vi "PPL_TRAJECTORY_EXECUTE_REL.vi"(8 "Init":bool, 9 "Max Wheel Speed M/S":dbl=2.5, 11 "Gyro Heading\nRAD":dbl) -> (0 "AtReference":bool, 1 "Position Error Ft":dbl, 2 "Right Speed Dmd M/S":dbl, 3 "Left Speed Dmd M/S":dbl)   [LabVIEW 2019]
uses:
  <vilib>/Rock Robotics/WPI/ThirdParty/MJansen/PathPlanner/TypeDef/PathPlannerTrajectory.ctl
  <vilib>/Rock Robotics/WPI/ThirdParty/MJansen/PathPlanner/TypeDef/PathPlannerTrajectoryState.ctl
  <vilib>/Rock Robotics/WPI/ThirdParty/JAS_Junk/TrajLib/TypeDef/TRANSLATION2D.ctl
  <vilib>/Rock Robotics/WPI/ThirdParty/JAS_Junk/TrajLib/TypeDef/ROTATION2D.ctl
  <vilib>/Rock Robotics/WPI/ThirdParty/MJansen/PathPlanner/TypeDef/PathPlannerPathConstraints.ctl
  <vilib>/Rock Robotics/WPI/ThirdParty/JAS_Junk/TrajLib/VI/Util_GetTime_U32.vi
  <vilib>/Rock Robotics/WPI/ThirdParty/JAS_Junk/TrajLib/Conv_Deg_Radians.vi
  <vilib>/Rock Robotics/WPI/ThirdParty/JAS_Junk/TrajLib/VI/DiffDrvOdom2_New.vi
  <vilib>/Rock Robotics/WPI/ThirdParty/JAS_Junk/TrajLib/VI/DiffDrvOdom2_Reset.vi
  <vilib>/Rock Robotics/WPI/ThirdParty/JAS_Junk/TrajLib/VI/DiffDrvOdom2_Update.vi
  <vilib>/Rock Robotics/WPI/ThirdParty/JAS_Junk/TrajLib/Rotation2d_GetRadians.vi
  <vilib>/Rock Robotics/SystemInterfaces/NetworkCommunication/NetComm_UsageReport_report.vi
  <vilib>/Rock Robotics/WPI/ThirdParty/JAS_Junk/TrajLib/Pose2d_getRotation.vi
  <vilib>/Rock Robotics/WPI/ThirdParty/JAS_Junk/TrajLib/Rotation2d_Minus.vi
  <vilib>/Rock Robotics/WPI/ThirdParty/JAS_Junk/TrajLib/Rotation2d_Plus.vi
  <vilib>/Rock Robotics/WPI/ThirdParty/JAS_Junk/TrajLib/Twist2d_Create.vi
  <vilib>/Rock Robotics/WPI/ThirdParty/JAS_Junk/TrajLib/Rotation2d_UnaryMinus.vi
  <vilib>/Rock Robotics/WPI/ThirdParty/JAS_Junk/TrajLib/Rotation2d_RotateBy.vi
  <vilib>/Rock Robotics/WPI/ThirdParty/JAS_Junk/TrajLib/Rotation2d_CreateXY.vi
  <vilib>/Rock Robotics/WPI/ThirdParty/JAS_Junk/TrajLib/Util_CalcDist.vi
  <vilib>/Rock Robotics/WPI/ThirdParty/JAS_Junk/TrajLib/VI/Util_GetTime_U64.vi
  PPL_TRAJECTORY_GLOBALS.vi
  Diff_Drive_System/PPL_DRIVE_GLOBALS.vi
  <vilib>/Rock Robotics/WPI/ThirdParty/JAS_Junk/TrajLib/Globals/Util_LibraryGlobals.vi
  <vilib>/Rock Robotics/WPI/ThirdParty/JAS_Junk/TrajLib/Pose2d_Exp.vi
  <vilib>/Rock Robotics/WPI/ThirdParty/JAS_Junk/TrajLib/Trajectory_Library.lvlib
  <vilib>/Rock Robotics/WPI/ThirdParty/MJansen/PathPlanner/PathPlanner24.lvlib
panel:
  out "PathPlannerTrajectory":T1 {"States"."TargetHolonomicRotation"."SIN" format="%13.4f"; "States"."TargetHolonomicRotation"."COS" format="%13.4f"; "States"."TargetHolonomicRotation"."VALUE" format="%13.4f"; "States"."Heading"."SIN" format="%13.4f"; "States"."Heading"."COS" format="%13.4f"; "States"."Heading"."VALUE" format="%13.4f"; "States"."PositionMeters"."Y" format="%14.3f"; "States"."PositionMeters"."X" format="%14.3f"}
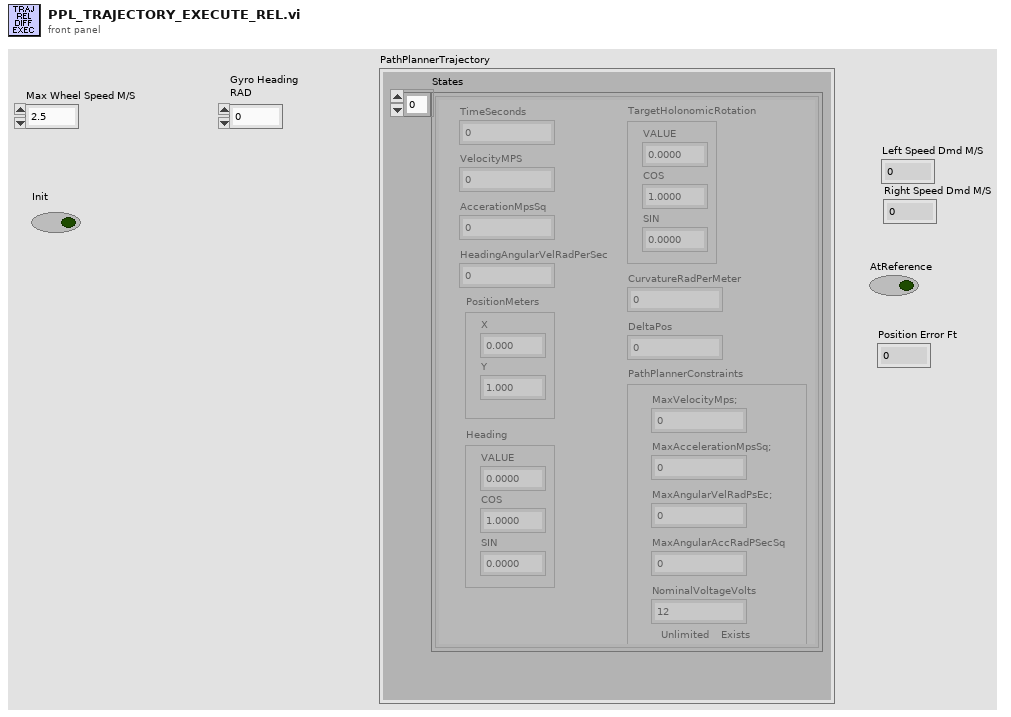
[diagram p1: front panel]
types:
  T1 = typedef "PathPlanner24.lvlib/PathPlannerTrajectory.ctl" = cluster{"States":T2[]}
  T2 = typedef "PathPlanner24.lvlib/PathPlannerTrajectoryState.ctl" = cluster{"TimeSeconds":dbl, "VelocityMPS":dbl, "AccerationMpsSq":dbl, "HeadingAngularVelRadPerSec":dbl, "PositionMeters":T3, "Heading":T4, "TargetHolonomicRotation":T4, "CurvatureRadPerMeter":dbl, "PathPlannerConstraints":T5, "DeltaPos":dbl}
  T3 = typedef "Trajectory_Library.lvlib/TRANSLATION2D.ctl" = cluster{"X":dbl, "Y":dbl}
  T4 = typedef "Trajectory_Library.lvlib/ROTATION2D.ctl" = cluster{"VALUE":dbl, "COS":dbl, "SIN":dbl}
  T5 = typedef "PathPlanner24.lvlib/PathPlannerPathConstraints.ctl" = cluster{"MaxVelocityMps;":dbl, "MaxAccelerationMpsSq;":dbl, "MaxAngularVelRadPsEc;":dbl, "MaxAngularAccRadPSecSq":dbl, "Exists":bool, "Unlimited":bool, "NominalVoltageVolts":dbl}
  T6 = typedef "Trajectory_Library.lvlib/POSE2D.ctl" = cluster{"TRANSLATION":T3, "ROTATION":T4}
  T7 = typedef "Trajectory_Library.lvlib/DIFF_DRIVE_KINEMATICS.ctl" = cluster{"TrackWidth_Meters":dbl}
  T8 = typedef "Trajectory_Library.lvlib/LTV_UNICYCLE_CONTROLLER_MODEL_PARAMS.CTL" = cluster{"Max linear ctrl effort M/S":dbl, "Max angular ctrl effort Rad/S":dbl, "Max Heading Meas Tol Rad":dbl, "Max X Pos Meas Tol M":dbl, "Max Y Pos Meas Tol M":dbl, "Max Linear Vel M/S":dbl}
  T9 = typedef "PathPlanner24.lvlib/PathPlannerCtrlLTVUnicycleConfig.ctl" = cluster{"Max Wheel Speed M/S":dbl, "Track Width M":dbl, "LTV_Unicycle_Ctrl_Model":T8, "LTV_Unicycle_Ctrl_Tolerance":T10}
  T10 = typedef "Trajectory_Library.lvlib/LTV_UNICYCLE_CONTROLLER_TOLERANCE.CTL" = cluster{"Max Heading Tolerance Rad":dbl, "Max X Tolerance M":dbl, "Max Y Tolerance M":dbl}
  T11 = typedef "Trajectory_Library.lvlib/LTV_UNICYCLE_CONTROLLER.ctl" = cluster{"States":i32, "Inputs":i32, "PoseError":T6, "PoseTolerance":T6, "Dt":dbl, "Enabled":bool, "LQR_K_Table":T12}
  T12 = typedef "Trajectory_Library.lvlib/FUNCTION_GENERATOR_MATRIX.ctl" = cluster{"Table Xs":dbl[], "Table Ys":variant[], "MinX":dbl, "MaxX":dbl, "ItemCount":i32, "Rows":i32, "Columns":i32}
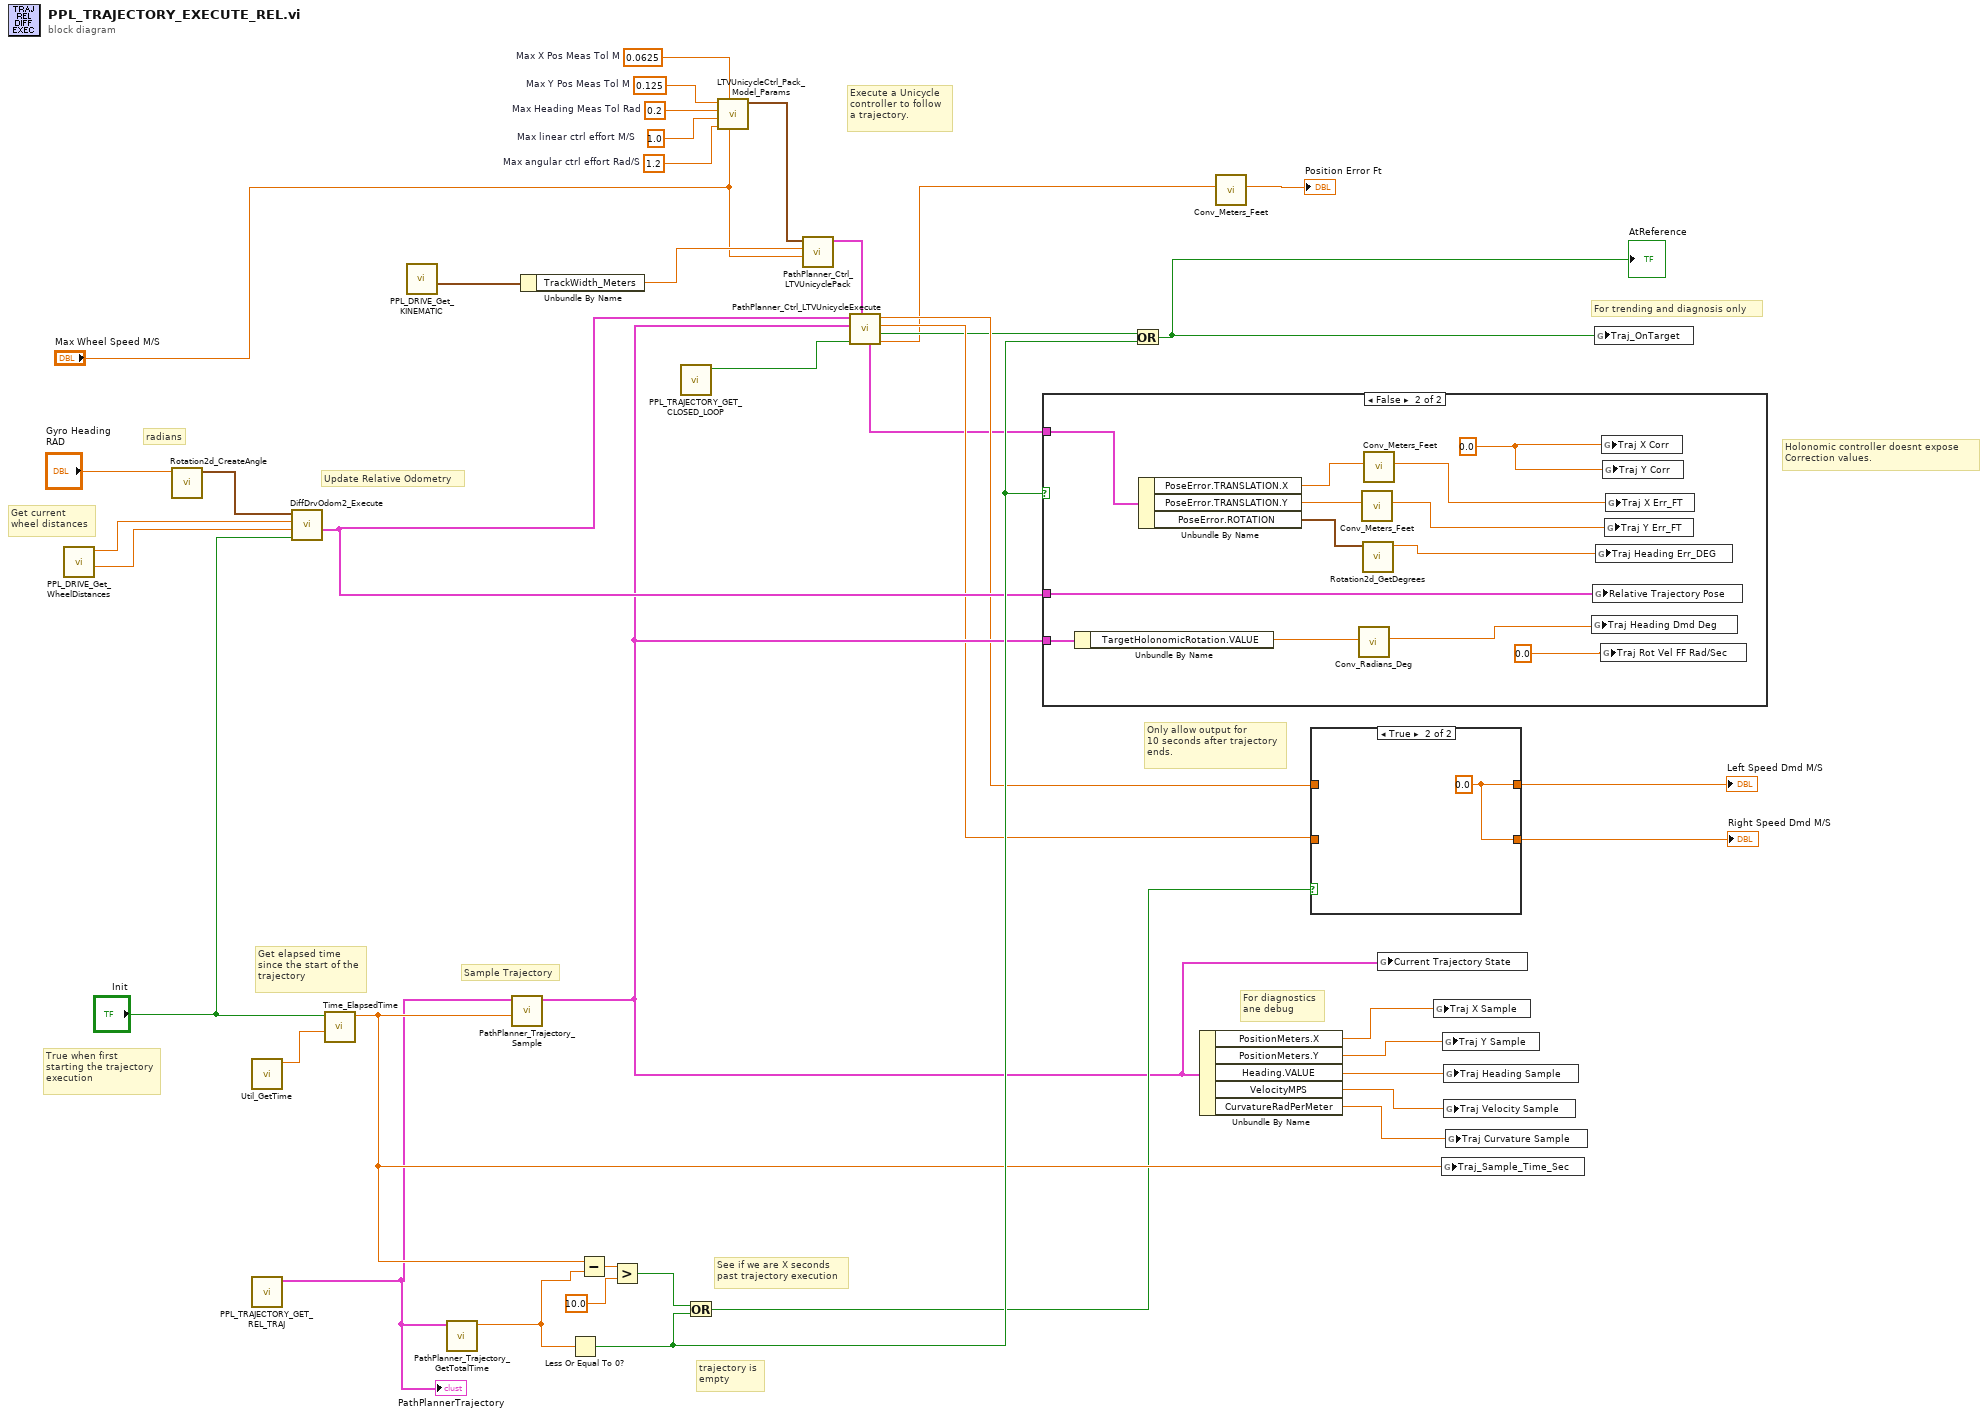
[diagram p0: block diagram]
diagram:
  w15 = 0.125  # Max Y Pos Meas Tol M
  w14 = 0.2  # Max Heading Meas Tol Rad
  w13 = 1.0  # Max linear ctrl effort M/S
  w12 = 1.2  # Max angular ctrl effort Rad/S
  w11 = 0.0625  # Max X Pos Meas Tol M
  # "Execute a Unicycle\ncontroller to follow\na trajectory."
  # "Get current \nwheel distances"
  # "Update Relative Odometry"
  # "radians"
  # "trajectory is \nempty"
  # "True when first\nstarting the trajectory\nexecution"
  # "Get elapsed time\nsince the start of the\ntrajectory"
  # "Holonomic controller doesnt expose\nCorrection values."
  # "For trending and diagnosis only"
  # "For diagnostics\nane debug"
  # "Sample Trajectory"
  # "See if we are X seconds \npast trajectory execution"
  # "Only allow output for\n10 seconds after trajectory\nends."
  n1 = call "PPL_DRIVE_Get_WheelDistances.vi"() -> ("Right Wheel Dist M"=w23:dbl, "Left Wheel Dist M"=w24:dbl)  [unwired: 10 in]
  n2 = call <vilib>:"Rotation2d_CreateAngle.vi"("Angle"="Gyro Heading\nRAD") -> ("ROTATION"=w26:T4)  [unwired: 10 in]
  n3 = call <vilib>:"Util_GetTime.vi"() -> ("FPGA_Time_Seconds"=w39:dbl)  [unwired: 9 in, 2 out]
  n4 = call "PPL_TRAJECTORY_GET_REL_TRAJ.vi"() -> ("Relative_Trajectory"=w28:T1)  [unwired: 11 in]
  "PathPlannerTrajectory" <- w28
  n5 = call <vilib>:"DiffDrvOdom2_Execute.vi"("Init / Reset"="Init", "Right Distance M"=w23, "Left Distance M"=w24, "Gyro Reading"=w26) -> ("Pose Meters"=w8:T6)  [unwired: 6 in, 1 out]
  n6 = call <vilib>:"Time_ElapsedTime.vi"("PassthroughTime_SEC"=w39, "Reset"="Init") -> ("Elapsed Time Sec"=w30:dbl)  [unwired: 9 in]
  n7 = call "PPL_DRIVE_Get_KINEMATIC.vi"() -> ("out DIFF_DRIVE_KINEMATICS"=w18:T7)  [unwired: 11 in]
  n8 = call <vilib>:"PathPlanner_Trajectory_GetTotalTime.vi"("PathPlannerTrajectory"=w28) -> ("TotalTimeSeconds"=w29:dbl)  [unwired: 10 in]
  n9 = call <vilib>:"PathPlanner_Trajectory_Sample.vi"("Time"=w30, "PathPlannerTrajectory"=w28) -> ("PathPlannerState"=w7:T2)  [unwired: 9 in]
  n10 = Unbundle By Name(w18) -> ("TrackWidth_Meters"=w10:dbl)
  n11 = Less Or Equal To 0?(x=w29) -> (x <= 0?=w31:bool)
  n12 = Subtract(x=w30, y=w29) -> (x-y=w41:dbl)
  n13 = Greater?(x=w41, y=10.0) -> (0:w33:bool)
  n14 = call "PPL_TRAJECTORY_GET_CLOSED_LOOP.vi"() -> ("AUTO_CLOSED_LOOP"=w9:bool)  [unwired: 11 in]
  n15 = Or(x=w33, y=w31) -> (x .or. y?=w20:bool)
  n16 = call <vilib>:"LTVUnicycleCtrl_Pack_Model_Params.vi"("Max Linear Vel M/S"="Max Wheel Speed M/S", "Max X Pos Meas Tol M"=w11, "Max angular ctrl effort Rad/S"=w12, "Max linear ctrl effort M/S"=w13, "Max Heading Meas Tol Rad"=w14, "Max Y Pos Meas Tol M"=w15) -> ("LTV_Unicycle_Ctrl_Model _Params"=w17:T8)  [unwired: 5 in]
  n17 = call <vilib>:"PathPlanner_Ctrl_LTVUnicyclePack.vi"("Max Speed M/S"="Max Wheel Speed M/S", "Track Width Meters"=w10, "LTV_Unicycle_Ctrl_Model"=w17) -> ("PathPlanner_Ctrl_LTVUnicycleConfig"=w16:T9)  [unwired: 8 in]
  n18 = call <vilib>:"PathPlanner_Ctrl_LTVUnicycleExecute.vi"("PathPlanner_Ctrl_LTVUnicycle_Config"=w16, "Enabled"=w9, "PathPlannerState"=w7, "Current Pose SI"=w8) -> ("Position Error M"=w2:dbl, "At Reference"=w3:bool, "Normalized Right Wheel Dmd M/S"=w4:dbl, "Normalized Left Wheel Dmd M/S"=w5:dbl, "out LTV_UNICYCLE_CONTROLLER"=w1:T11)  [unwired: 3 in]
  n19 = case shown="False" w31 {
    tunnel: w8 -> [_ w45]
    tunnel: w7 -> [_ w48]
    tunnel: w1 -> [_ w42]
    frame True {
    }
    frame False {
      w54 = 0.0 ("Y Corr")
      n20 = Unbundle By Name(w48) -> ("TargetHolonomicRotation.VALUE"=w47:dbl)
      n21 = Unbundle By Name(w42) -> ("PoseError.TRANSLATION.X"=w50:dbl, "PoseError.TRANSLATION.Y"=w49:dbl, "PoseError.ROTATION"=w43:T4)
      n22 = call <vilib>:"Conv_Radians_Deg.vi"("Radians"=w47) -> ("Degrees"=w46:dbl)  [unwired: 10 in]
      n23 = call <vilib>:"Conv_Meters_Feet.vi"("Meters"=w49) -> ("Feet"=w53:dbl)  [unwired: 10 in]
      n24 = call <vilib>:"Rotation2d_GetDegrees.vi"("in ROTATION"=w43) -> ("AngleDegrees"=w44:dbl)  [unwired: 10 in]
      n25 = call <vilib>:"Conv_Meters_Feet.vi"("Meters"=w50) -> ("Feet"=w52:dbl)  [unwired: 10 in]
      n26 = global write "PPL_TRAJECTORY_GLOBALS.vi" "Traj Heading Dmd Deg"(w46) -> ()
      n27 = global write "PPL_TRAJECTORY_GLOBALS.vi" "Relative Trajectory Pose"(w45) -> ()
      n28 = global write "PPL_TRAJECTORY_GLOBALS.vi" "Traj Heading Err_DEG"(w44) -> ()
      n29 = global write "PPL_TRAJECTORY_GLOBALS.vi" "Traj Rot Vel FF Rad/Sec"(0.0 ("Traj Heading Dmd Deg")) -> ()
      n30 = global write "PPL_TRAJECTORY_GLOBALS.vi" "Traj X Corr"(w54) -> ()
      n31 = global write "PPL_TRAJECTORY_GLOBALS.vi" "Traj Y Corr"(w54) -> ()
      n32 = global write "PPL_TRAJECTORY_GLOBALS.vi" "Traj Y Err_FT"(w53) -> ()
      n33 = global write "PPL_TRAJECTORY_GLOBALS.vi" "Traj X Err_FT"(w52) -> ()
    }
  }
  n34 = Or(x=w3, y=w31) -> (x .or. y?=w32:bool)
  "AtReference" <- w32
  n35 = Unbundle By Name(w7) -> ("PositionMeters.X"=w38:dbl, "PositionMeters.Y"=w37:dbl, "Heading.VALUE"=w36:dbl, "VelocityMPS"=w35:dbl, "CurvatureRadPerMeter"=w34:dbl)
  n36 = call <vilib>:"Conv_Meters_Feet.vi"("Meters"=w2) -> ("Feet"=→"Position Error Ft":dbl)  [unwired: 10 in]
  n37 = case shown="True" w20 {
    tunnel: w5 -> [w56 _]
    tunnel: [w56 w57] -> w22
    tunnel: w4 -> [w55 _]
    tunnel: [w55 w57] -> w21
    frame False {
    }
    frame True {
      w57 = 0.0 ("vX")
    }
  }
  "Left Speed Dmd M/S" <- w22
  "Right Speed Dmd M/S" <- w21
  n38 = global write "PPL_TRAJECTORY_GLOBALS.vi" "Current Trajectory State"(w7) -> ()
  n39 = global write "PPL_TRAJECTORY_GLOBALS.vi" "Traj X Sample"(w38) -> ()
  n40 = global write "PPL_TRAJECTORY_GLOBALS.vi" "Traj_Sample_Time_Sec"(w30) -> ()
  n41 = global write "PPL_TRAJECTORY_GLOBALS.vi" "Traj Y Sample"(w37) -> ()
  n42 = global write "PPL_TRAJECTORY_GLOBALS.vi" "Traj Heading Sample"(w36) -> ()
  n43 = global write "PPL_TRAJECTORY_GLOBALS.vi" "Traj Velocity Sample"(w35) -> ()
  n44 = global write "PPL_TRAJECTORY_GLOBALS.vi" "Traj Curvature Sample"(w34) -> ()
  n45 = global write "PPL_TRAJECTORY_GLOBALS.vi" "Traj_OnTarget"(w32) -> ()
